vi "VIH Dialog - ProjectType.vi"(7 "Title":string="New Project") -> (0 "OK out":bool, 3 "Project Type out":enum32{"Default", "JSBased"}(ring) caption="Project type")   [LabVIEW 2014]
doc: "::: VI Helpeks :::\nCopyright (c) 2000-2026 Konstantin Shifershteyn. All rights reserved."
panel:
  in  "OK":bool
  in  "Cancel":bool
  in  "Project Type":enum32{"Default", "JSBased"}(radio) caption="Project type"
  # "Select Project Type"
  # "If you select Default project type, the project's Master Rule will be configured for generating help files in pure HTML format with flat layout."
  # "If you select JavaScript based project type, the project's Master Rule will be configured for generating help files that use JavaScript for providing additional features like LabVIEW Help."
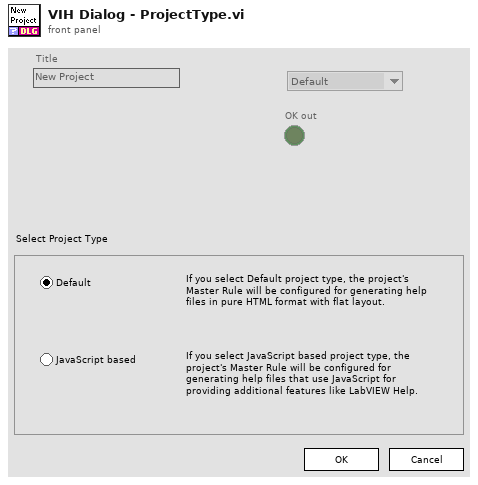
[diagram p1: front panel]
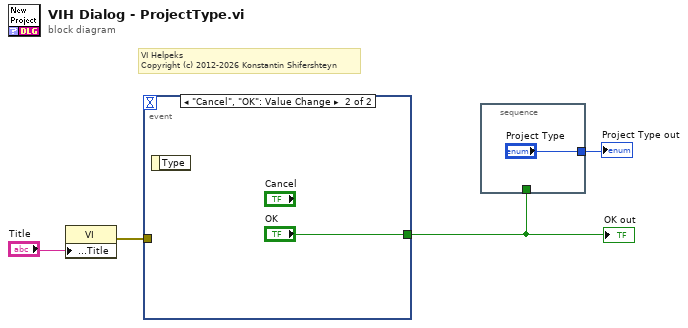
[diagram p0: block diagram]
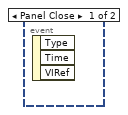
[diagram p2: hidden frame]
diagram:
  # "VI Helpeks\nCopyright (c) 2012-2026 Konstantin Shifershteyn"
  n1 = property class="VI"("Front Panel.Title"="Title") -> (error out=w1:errorcluster)  [unwired: 2 in, 1 out]
  n2 = event shown="[1] \"Cancel\", \"OK\": Value Change" {
    selector: _ -> [_ _]
    dyn-events: _ -> [_ _]
    timeout: _ -> [_ _]
    tunnel: [_ "OK"] -> w4
    tunnel: w1 -> [_ _]
    event Panel Close {
      n3 = event-data() -> ()  [unwired: 1 in, 3 out]
    }
    event "Cancel", "OK": Value Change {
      n4 = event-data() -> ()  [unwired: 1 in, 1 out]
    }
  }
  "OK out" <- w4
  n5 = stacked-sequence {
    tunnel: w4 -> [_]
    tunnel: ["Project Type"] -> w3
    frame #0 {
    }
  }
  "Project Type out" <- w3
